vi "ErrBool B.vi"(11 "error in":errorcluster) -> ()   [LabVIEW 2026]
doc: "Probe: an error cluster wired straight into a While Loop's stop terminal."
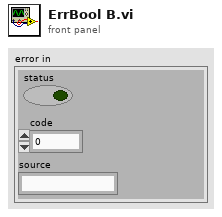
[diagram p1: front panel]
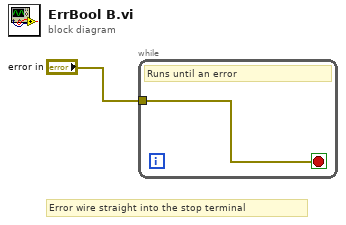
[diagram p0: block diagram]
diagram:
  # "Error wire straight into the stop terminal"
  n1 = while {
    tunnel: "error in" -> [w2]
    stop <- w2 stop-if-true
    # "Runs until an error"
  }
